vi "Test MQTT-6.0.0-4.vi"(8 "error in (no error)":errorcluster, 11 "Connection":refnum<class "Connection.lvclass">) -> (0 "error out":errorcluster, 3 "Connection":refnum<class "Connection.lvclass">)   [LabVIEW 2013]
uses:
  <vilib>/LabVIEW Open Source Project/Connection/Connection/Connection.lvclass
  <vilib>/LabVIEW Open Source Project/Connection/Connection.Websockets/Connection.WS.lvclass
  <vilib>/LabVIEW Open Source Project/Connection/Connection.Websockets/Connection.WS.lvclass/Connection.WS.ctl
  <vilib>/addons/_JKI Toolkits/Caraya/classes/Test/Test.lvclass
  <vilib>/addons/_JKI Toolkits/Caraya/classes/Assert/Assert.lvclass
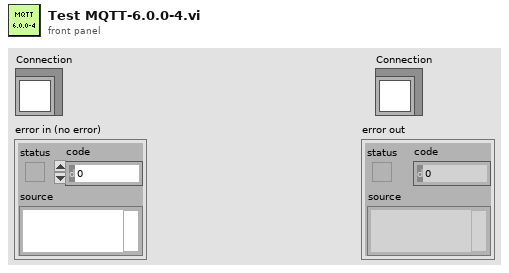
[diagram p1: front panel]
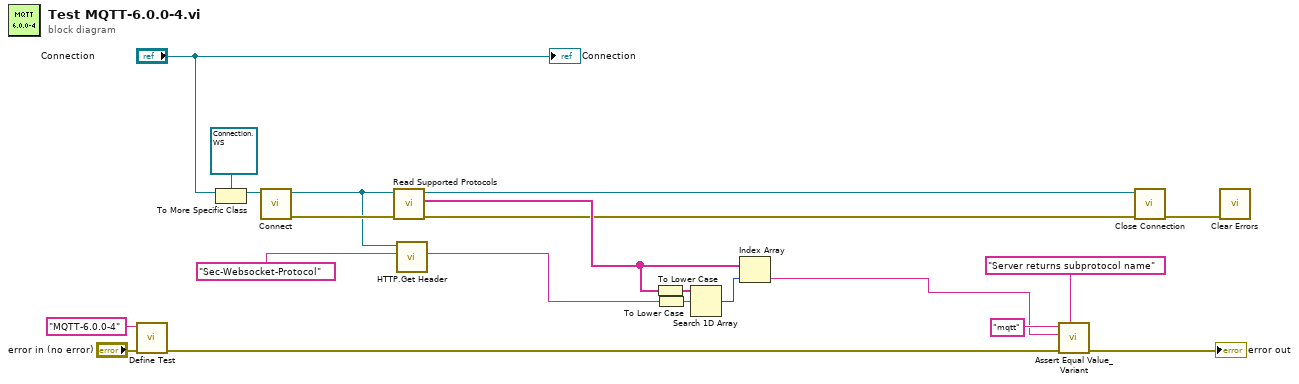
[diagram p0: block diagram]
diagram:
  n1 = call <vilib>:"Define Test.vi"("error in (no error)"="error in (no error)", "Label (VI Title)"="MQTT-6.0.0-4") -> ("error out"=w18:errorcluster)  [unwired: 9 in]
  n2 = To More Specific Class(target class=refnum<class "Connection.WS.lvclass"> refnum ("Connection.WS in"), reference="Connection") -> (specific class reference=w15:refnum<class "Connection.WS.lvclass">)  [unwired: 1 in, 1 out]
  n3 = call <vilib>:"Connect.vi"("Connection in"=w15) -> ("error out"=w7:errorcluster, "Connection out"=w4:refnum<class "Connection.WS.lvclass">)  [unwired: 9 in]
  n4 = call <vilib>:"Read Supported Protocols.vi"("error in (no error)"=w7, "Connection.WS in"=w4) -> ("error out"=w6:errorcluster, "Supported Protocols"=w9:string[], "Connection.WS out"=w8:refnum<class "Connection.WS.lvclass">)  [unwired: 6 in, 1 out]
  n5 = call <vilib>:"HTTP.Get Header.vi"("Header Name"="Sec-Websocket-Protocol" ("name"), "Connection.WS in"=w4) -> ("Value"=w2:string)  [unwired: 6 in, 3 out]
  n6 = To Lower Case(string=w9) -> (all lower case string=w12:string[])
  n7 = To Lower Case(string=w2) -> (all lower case string=w11:string)
  n8 = Search 1D Array(1D array=w12, element=w11) -> (index of element=w10:i32)  [unwired: 1 in]
  n9 = Index Array(array=w9, index=w10) -> (element=w5:string)
  n10 = call <vilib>:"Assert Equal Value_Variant.vi"("Label"="Server returns subprotocol name", "error in (no error)"=w18, "Y"=w5, "X"="mqtt") -> ("error out"=→"error out":errorcluster)  [unwired: 7 in]
  n11 = call <vilib>:"Close Connection.vi"("error in (no error)"=w6, "Connection in"=w8) -> ("error out"=w14:errorcluster)  [unwired: 8 in, 1 out]
  n12 = call <vilib>:"Clear Errors.vi"("error in (no error)"=w14) -> ()  [unwired: 6 in, 1 out]
  "Connection" <- "Connection"
